vi "Actividad 1 Interfaz Labview.vi"() -> ()   [LabVIEW 2026]
panel:
  out ">10°C":bool
  out "< 80°C":bool
  out "?":string
  out "?":string
  out "Celcius (°C)":dbl(slide) scale=-150.0..150.0
  in  "stop":bool
  out "Kelvin (°K)":dbl(slide) scale=-150.0..800.0
  out "Farenheit (°F)":dbl(slide) scale=-150.0..500.0
  in  "SLIDER":dbl(slide) scale=-100.0..200.0
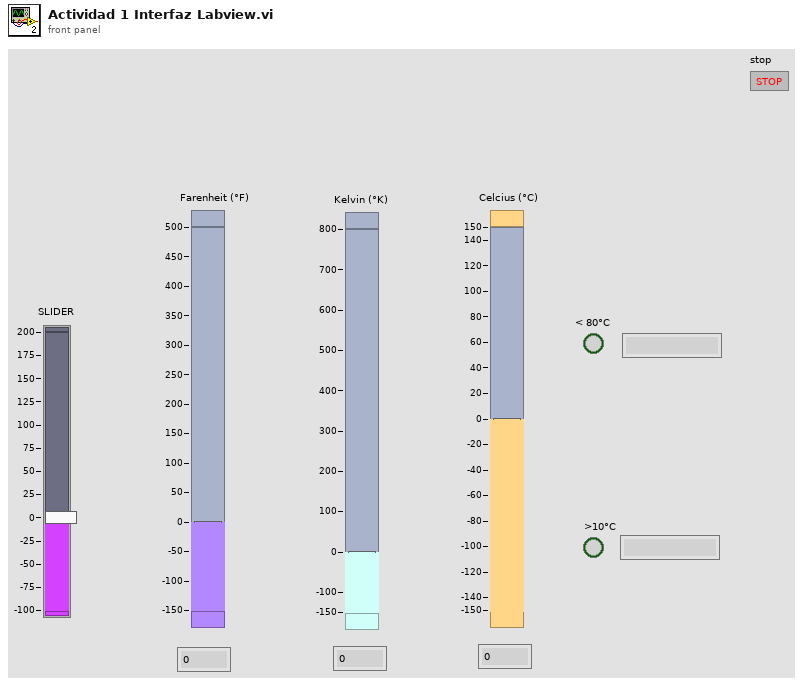
[diagram p1: front panel]
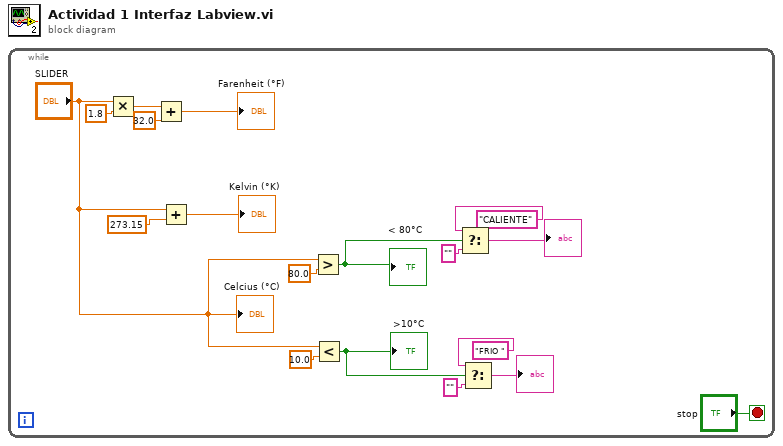
[diagram p0: block diagram]
diagram:
  n1 = while {
    stop <- "stop" stop-if-true
    n2 = Multiply(x="SLIDER", y=1.8) -> (x*y=w17:dbl)
    n3 = Add(x=w17, y=32.0) -> (x+y=→"Farenheit (°F)":dbl)
    n4 = Add(x="SLIDER", y=273.15) -> (x+y=→"Kelvin (°K)":dbl)
    n5 = Greater?(x="SLIDER", y=80.0) -> (0:w3:bool)
    "< 80°C" <- w3
    n6 = Less?(x="SLIDER", y=10.0) -> (x < y?=w2:bool)
    ">10°C" <- w2
    n7 = Select(t="CALIENTE", s=w3, f="") -> (s? t:f=→"?":string)
    n8 = Select(t="FRIO ", s=w2, f="") -> (s? t:f=→"?":string)
    "Celcius (°C)" <- "SLIDER"
  }
